vi "Test Deserialize Enum.vi"(8 "error in (no error)":errorcluster) -> (0 "error out":errorcluster)   [LabVIEW 2013]
uses:
  src/Deserializer/JSON Deserializer/JSON Deserializer.lvclass
  <vilib>/addons/_JKI Toolkits/Caraya/classes/Test/Test.lvclass
  <vilib>/addons/_JKI Toolkits/Caraya/classes/Assert/Assert.lvclass
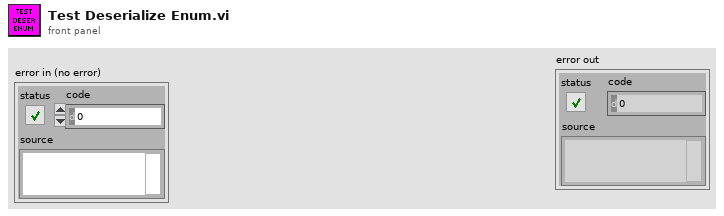
[diagram p1: front panel]
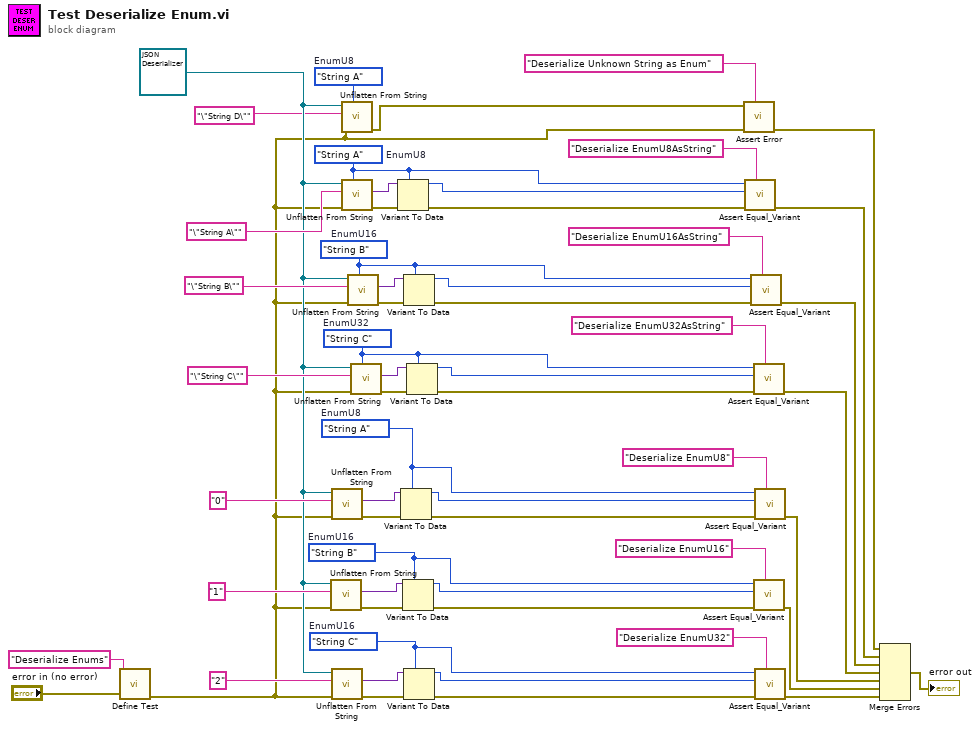
[diagram p0: block diagram]
diagram:
  w7 = enum8{"String A", "String B", "String C"}."String A"  # EnumU8
  w14 = enum32{"String A", "String B", "String C"}."String C"  # EnumU32
  w25 = enum16{"String A", "String B", "String C"}."String B"  # EnumU16
  w33 = enum16{"String A", "String B", "String C"}."String B"  # EnumU16
  w34 = enum32{"String A", "String B", "String C"}."String C"  # EnumU16
  w8 = enum8{"String A", "String B", "String C"}."String A"  # EnumU8
  w9 = enum8{"String A", "String B", "String C"}."String A"  # EnumU8
  w6 = refnum<class "JSON Deserializer.lvclass"> refnum ("JKI JSON Serialization.lvlib:JSON Deserializer.lvclass")
  n1 = call <vilib>:"Define Test.vi"("error in (no error)"="error in (no error)", "Label (VI Title)"="Deserialize Enums") -> ("error out"=w1:errorcluster)  [unwired: 9 in]
  n2 = call-dynamic "Unflatten From String.vi"("error in (no error)"=w1, "String"="1", "Deserializer in"=w6) -> ("error out"=w27:errorcluster, "Variant"=w30:variant)  [unwired: 6 in, 1 out]
  n3 = call-dynamic "Unflatten From String.vi"("error in (no error)"=w1, "String"="0", "Deserializer in"=w6) -> ("error out"=w44:errorcluster, "Variant"=w40:variant)  [unwired: 6 in, 1 out]
  n4 = call-dynamic "Unflatten From String.vi"("error in (no error)"=w1, "String"="2", "Deserializer in"=w6) -> ("error out"=w46:errorcluster, "Variant"=w38:variant)  [unwired: 6 in, 1 out]
  n5 = call-dynamic "Unflatten From String.vi"("Type and Defaults"=w7, "error in (no error)"=w1, "String"="\"String D\"", "Deserializer in"=w6) -> ("error out"=w3:errorcluster)  [unwired: 5 in, 2 out]
  n6 = call-dynamic "Unflatten From String.vi"("Type and Defaults"=w9, "error in (no error)"=w1, "String"="\"String A\"", "Deserializer in"=w6) -> ("error out"=w50:errorcluster, "Variant"=w51:variant)  [unwired: 5 in, 1 out]
  n7 = call-dynamic "Unflatten From String.vi"("Type and Defaults"=w25, "error in (no error)"=w1, "String"="\"String B\"", "Deserializer in"=w6) -> ("error out"=w21:errorcluster, "Variant"=w20:variant)  [unwired: 5 in, 1 out]
  n8 = call-dynamic "Unflatten From String.vi"("Type and Defaults"=w14, "error in (no error)"=w1, "String"="\"String C\"", "Deserializer in"=w6) -> ("error out"=w18:errorcluster, "Variant"=w19:variant)  [unwired: 5 in, 1 out]
  n9 = Variant To Data(error in=w50, type=w9, Variant=w51) -> (data=w47:enum8{"String A", "String B", "String C"}, error out=w48:errorcluster)
  n10 = Variant To Data(error in=w44, type=w8, Variant=w40) -> (data=w35:enum8{"String A", "String B", "String C"}, error out=w41:errorcluster)
  n11 = Variant To Data(error in=w27, type=w33, Variant=w30) -> (data=w32:enum16{"String A", "String B", "String C"}, error out=w29:errorcluster)
  n12 = Variant To Data(error in=w21, type=w25, Variant=w20) -> (data=w24:enum16{"String A", "String B", "String C"}, error out=w23:errorcluster)
  n13 = Variant To Data(error in=w46, type=w34, Variant=w38) -> (data=w36:enum32{"String A", "String B", "String C"}, error out=w39:errorcluster)
  n14 = Variant To Data(error in=w18, type=w14, Variant=w19) -> (data=w15:enum32{"String A", "String B", "String C"}, error out=w16:errorcluster)
  n15 = call <vilib>:"Assert Error.vi"("Label"="Deserialize Unknown String as Enum", "error in (no error)"=w1, "Error?"=w3) -> ("error out"=w4:errorcluster)  [unwired: 8 in]
  n16 = call <vilib>:"Assert Equal_Variant.vi"("Label"="Deserialize EnumU8AsString", "error in (no error)"=w48, "Y"=w47, "X"=w9) -> ("error out"=w26:errorcluster)  [unwired: 7 in]
  n17 = call <vilib>:"Assert Equal_Variant.vi"("Label"="Deserialize EnumU16AsString", "error in (no error)"=w23, "Y"=w24, "X"=w25) -> ("error out"=w13:errorcluster)  [unwired: 7 in]
  n18 = call <vilib>:"Assert Equal_Variant.vi"("Label"="Deserialize EnumU32AsString", "error in (no error)"=w16, "Y"=w15, "X"=w14) -> ("error out"=w12:errorcluster)  [unwired: 7 in]
  n19 = call <vilib>:"Assert Equal_Variant.vi"("Label"="Deserialize EnumU16", "error in (no error)"=w29, "Y"=w32, "X"=w33) -> ("error out"=w53:errorcluster)  [unwired: 7 in]
  n20 = call <vilib>:"Assert Equal_Variant.vi"("Label"="Deserialize EnumU8", "error in (no error)"=w41, "Y"=w35, "X"=w8) -> ("error out"=w55:errorcluster)  [unwired: 7 in]
  n21 = call <vilib>:"Assert Equal_Variant.vi"("Label"="Deserialize EnumU32", "error in (no error)"=w39, "Y"=w36, "X"=w34) -> ("error out"=w56:errorcluster)  [unwired: 7 in]
  n22 = Merge Errors(w4, w26, w13, w12, w55, w53, w56) -> (→"error out":errorcluster)
